vi "FuncVI_Sub - Format to string.vi"(5 "InstanceRef":T2, 7 "format error enabled":bool, 9 "arg list":T1[](array[typedef]) {"num" format="%.2f"}) -> (0 "error out":bool, 3 "result":T1 {"num" format="%.2f"})   [LabVIEW 2021]
doc: "::: CalcExpress Toolkit :::\nCopyright (c) 2000-2026 Konstantin Shifershteyn. All rights reserved."
uses:
  cetypes.llb/CalcExpress Function Argument Info.ctl
  cetypes.llb/CalcExpress Instance RefNum.ctl
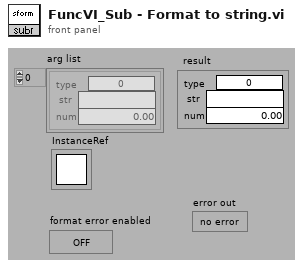
[diagram p1: front panel]
types:
  T1 = typedef "CalcExpress Function Argument Info.ctl" = cluster{"type":u32, "str":string, "num":dbl}
  T2 = typedef "CalcExpress Instance RefNum.ctl" = refnum<k1>
  T3 = enum32{"String", "DBL Number", "identifier", "1D Array of DBL", "2D Array of DBL", "CDB Number", "1D Array of CDB", "2D Array of CDB", "1D Array of String", "2D Array of String", "Unknown data type"}
  T4 = cluster{"type":enum32{"String", "DBL Number", "identifier", "1D Array of DBL", "2D Array of DBL", "CDB Number", "1D Array of CDB", "2D Array of CDB", "1D Array of String", "2D Array of String", "Unknown data type"}, string, "return value":dbl}
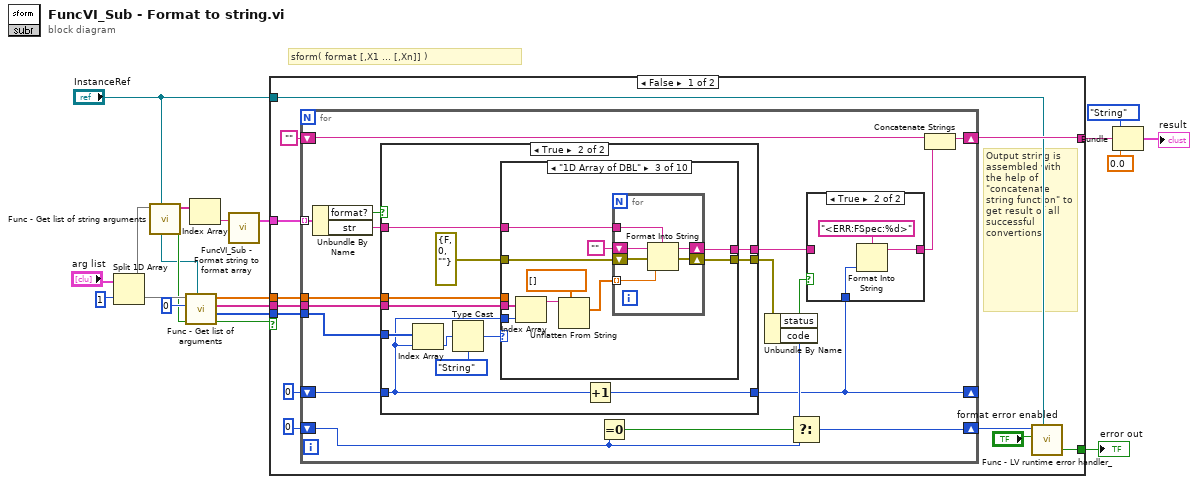
[diagram p0: block diagram]
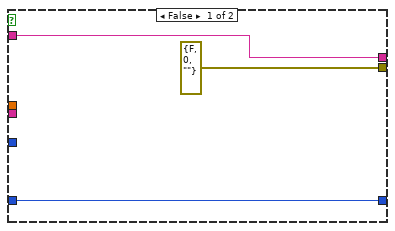
[diagram p3: hidden frame]
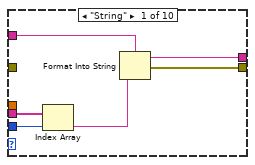
[diagram p4: hidden frame]
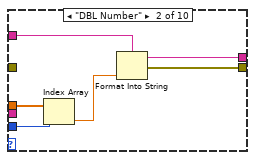
[diagram p5: hidden frame]
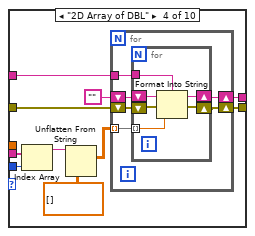
[diagram p6: hidden frame]
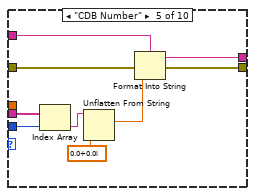
[diagram p7: hidden frame]
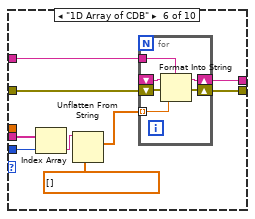
[diagram p8: hidden frame]
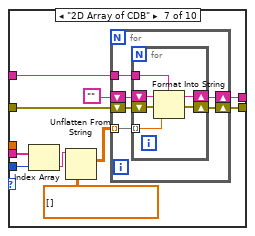
[diagram p9: hidden frame]
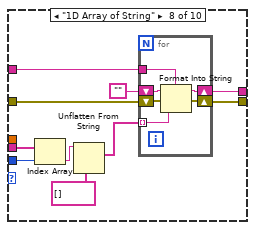
[diagram p10: hidden frame]
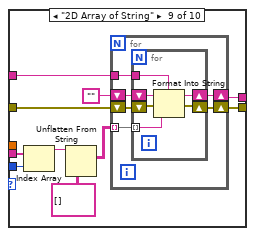
[diagram p11: hidden frame]
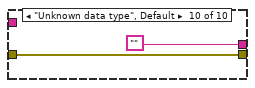
[diagram p12: hidden frame]
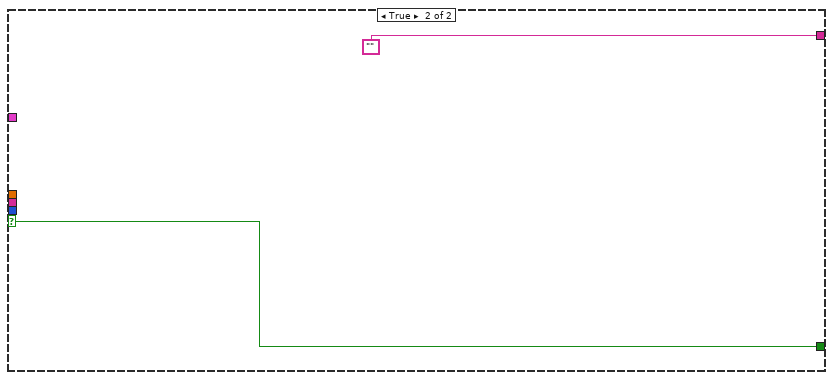
[diagram p13: hidden frame]
diagram:
  # "sform( format [,X1 ... [,Xn]] )"
  n1 = Split 1D Array(array="arg list", index=1) -> (first subarray=w17:T1[], second subarray=w16:T1[])
  n2 = call "Func - Get list of string arguments.vi"("InstanceRef"="InstanceRef", "arg list"=w17) -> ("error out"=w7:bool, "val list"=w5:string[])  [unwired: 6 in]
  n3 = call "Func - Get list of arguments.vi"("InstanceRef"="InstanceRef", "error in"=w7, "min arg num"=0 ("min args num"), "arg list"=w16) -> ("error out"=w6:bool, "type list"=w13:u32[], "str list"=w14:string[], "num list"=w2:dbl[])  [unwired: 4 in]
  n4 = Index Array(array=w5) -> (element=w4:string)  [unwired: 1 in]
  n5 = call "FuncVI_Sub - Format string to format array.vi"("format string"=w4) -> ("formats"=w3:cluster{"str":string, "format?":bool}[])  [unwired: 1 in, 1 out]
  n6 = case shown="False" w6 {
    selector: w6 -> [_ w205]
    tunnel: w2 -> [w31 _]
    tunnel: w14 -> [w30 _]
    tunnel: w13 -> [w28 _]
    tunnel: [w23 w205] -> w12
    tunnel: [w29 "" ("Empty String Constant")] -> w10
    tunnel: w3 -> [w25 _]
    tunnel: "InstanceRef" -> [w21 _]
    frame False {
      # "Output string is assembled with the help of \"concatenate string function\" to get result of all successful convertions."
      n7 = for {
        shift-right: [w39] -> w29
        shift-left: "" ("Empty String Constant") -> [w38]
        tunnel: w31 -> [w49]
        tunnel: w30 -> [w48]
        tunnel: w28 -> [w47]
        tunnel: w25 -> [w46] mode=indexing
        shift-right: [w34] -> _
        shift-left: 0 -> [w43]
        shift-right: [w40] -> w20
        shift-left: 0 -> [w41]
        n8 = Unbundle By Name(w46) -> ("format?"=w44:bool, "str"=w45:string)
        n9 = case shown="True" w44 {
          tunnel: w49 -> [_ w68]
          tunnel: w48 -> [_ w67]
          tunnel: w47 -> [_ w63]
          tunnel: [errorcluster {"status"=FALSE, "code"=0, "source"=""} ("error IO") w66] -> w42
          tunnel: w45 -> [w54 w65]
          tunnel: w43 -> [w56 w61]
          tunnel: [w56 w64] -> w34
          tunnel: [w54 w59] -> w33
          frame False {
          }
          frame True {
            n10 = Index Array(array=w63, index=w61) -> (element=w62:u32)
            n11 = Type Cast(type=T3."String", x=w62) -> (*(type *) &x=w58:T3)
            n12 = case shown="\"1D Array of DBL\"" w58 {
              tunnel: w68 -> [_ w77 _ _ _ _ _ _ _ _]
              tunnel: w67 -> [w74 _ w84 w99 w123 w136 w152 w174 w185 _]
              tunnel: [w73 w80 w86 w101 w127 w131 w147 w169 w186 "" ("Empty String Constant")] -> w59
              tunnel: [w72 w79 w88 w102 w126 w133 w148 w171 w187 w204] -> w66
              tunnel: w65 -> [w71 w78 w82 w104 w125 w128 w144 w168 w182 _]
              tunnel: errorcluster {"status"=FALSE, "code"=0, "source"=""} ("error IO") -> [_ _ w89 w103 w124 w134 w149 w172 w188 w204]
              tunnel: w61 -> [w69 w76 w85 w98 w119 w129 w145 w166 w184 _]
              frame "String" {
                n13 = Index Array(array=w74, index=w69) -> (element=w70:string)
                n14 = Format Into String(format string=w71, w70) -> (resulting string=w73:string, error out=w72:errorcluster)  [unwired: 2 in]
              }
              frame "DBL Number" {
                n15 = Index Array(array=w77, index=w76) -> (element=w75:dbl)
                n16 = Format Into String(format string=w78, w75) -> (resulting string=w80:string, error out=w79:errorcluster)  [unwired: 2 in]
              }
              frame "1D Array of DBL" {
                n17 = Index Array(array=w84, index=w85) -> (element=w83:string)
                n18 = Unflatten From String(type=dbl[] [] ("num list"), binary string=w83) -> (value=w87:dbl[])  [unwired: 3 in, 2 out]
                n19 = for {
                  tunnel: w87 -> [w96] mode=indexing
                  shift-right: [w93] -> w86
                  shift-left: "" ("Empty String Constant") -> [w92]
                  shift-right: [w94] -> w88
                  shift-left: w89 -> [w95]
                  tunnel: w82 -> [w91]
                  n20 = Format Into String(format string=w91, initial string=w92, error in=w95, w96) -> (resulting string=w93:string, error out=w94:errorcluster)
                }
              }
              frame "2D Array of DBL" {
                n21 = Index Array(array=w99, index=w98) -> (element=w100:string)
                n22 = Unflatten From String(type=dbl[][] [] ("num list"), binary string=w100) -> (value=w105:dbl[][])  [unwired: 3 in, 2 out]
                n23 = for {
                  tunnel: w105 -> [w112] mode=indexing
                  tunnel: w104 -> [w111]
                  shift-right: [w109] -> w102
                  shift-left: w103 -> [w110]
                  shift-right: [w108] -> w101
                  shift-left: "" ("Empty String Constant") -> [w107]
                  n24 = for {
                    tunnel: w112 -> [w118] mode=indexing
                    shift-right: [w114] -> w108
                    shift-left: w107 -> [w113]
                    shift-right: [w116] -> w109
                    shift-left: w110 -> [w117]
                    tunnel: w111 -> [w115]
                    n25 = Format Into String(format string=w115, initial string=w113, error in=w117, w118) -> (resulting string=w114:string, error out=w116:errorcluster)
                  }
                }
              }
              frame "CDB Number" {
                n26 = Index Array(array=w123, index=w119) -> (element=w120:string)
                n27 = Unflatten From String(type=cdb 0.0+0.0i, binary string=w120) -> (value=w122:cdb)  [unwired: 3 in, 2 out]
                n28 = Format Into String(format string=w125, error in=w124, w122) -> (resulting string=w127:string, error out=w126:errorcluster)  [unwired: 1 in]
              }
              frame "1D Array of CDB" {
                n29 = Index Array(array=w136, index=w129) -> (element=w130:string)
                n30 = Unflatten From String(type=cdb[] [] ("num list"), binary string=w130) -> (value=w132:cdb[])  [unwired: 3 in, 2 out]
                n31 = for {
                  tunnel: w132 -> [w142] mode=indexing
                  shift-right: [w138] -> w131
                  shift-left: _ -> [w139]
                  shift-right: [w140] -> w133
                  shift-left: w134 -> [w141]
                  tunnel: w128 -> [w137]
                  n32 = Format Into String(format string=w137, initial string=w139, error in=w141, w142) -> (resulting string=w138:string, error out=w140:errorcluster)
                }
              }
              frame "2D Array of CDB" {
                n33 = Index Array(array=w152, index=w145) -> (element=w146:string)
                n34 = Unflatten From String(type=cdb[][] [] ("num list"), binary string=w146) -> (value=w150:cdb[][])  [unwired: 3 in, 2 out]
                n35 = for {
                  tunnel: w150 -> [w158] mode=indexing
                  shift-right: [w156] -> w148
                  shift-left: w149 -> [w157]
                  shift-right: [w155] -> w147
                  shift-left: "" ("Empty String Constant") -> [w154]
                  tunnel: w144 -> [w153]
                  n36 = for {
                    tunnel: w158 -> [w164] mode=indexing
                    shift-right: [w161] -> w155
                    shift-left: w154 -> [w160]
                    shift-right: [w162] -> w156
                    shift-left: w157 -> [w163]
                    tunnel: w153 -> [w159]
                    n37 = Format Into String(format string=w159, initial string=w160, error in=w163, w164) -> (resulting string=w161:string, error out=w162:errorcluster)
                  }
                }
              }
              frame "1D Array of String" {
                n38 = Index Array(array=w174, index=w166) -> (element=w167:string)
                n39 = Unflatten From String(type=string[] [] ("num list"), binary string=w167) -> (value=w170:string[])  [unwired: 3 in, 2 out]
                n40 = for {
                  tunnel: w170 -> [w180] mode=indexing
                  shift-right: [w176] -> w169
                  shift-left: "" ("Empty String Constant") -> [w177]
                  shift-right: [w178] -> w171
                  shift-left: w172 -> [w179]
                  tunnel: w168 -> [w175]
                  n41 = Format Into String(format string=w175, initial string=w177, error in=w179, w180) -> (resulting string=w176:string, error out=w178:errorcluster)
                }
              }
              frame "2D Array of String" {
                n42 = Index Array(array=w185, index=w184) -> (element=w183:string)
                n43 = Unflatten From String(type=string[][] [] ("num list"), binary string=w183) -> (value=w189:string[][])  [unwired: 3 in, 2 out]
                n44 = for {
                  tunnel: w189 -> [w196] mode=indexing
                  shift-right: [w194] -> w187
                  shift-left: w188 -> [w195]
                  shift-right: [w193] -> w186
                  shift-left: "" ("Empty String Constant") -> [w192]
                  tunnel: w182 -> [w191]
                  n45 = for {
                    tunnel: w196 -> [w202] mode=indexing
                    shift-right: [w199] -> w193
                    shift-left: w192 -> [w198]
                    shift-right: [w200] -> w194
                    shift-left: w195 -> [w201]
                    tunnel: w191 -> [w197]
                    n46 = Format Into String(format string=w197, initial string=w198, error in=w201, w202) -> (resulting string=w199:string, error out=w200:errorcluster)
                  }
                }
              }
              frame "Unknown data type", Default {
              }
            }
            n47 = Increment(x=w61) -> (x+1=w64:i32)
          }
        }
        n48 = Equal To 0?(x=w41) -> (x = 0?=w37:bool)
        n49 = Unbundle By Name(w42) -> ("status"=w35:bool, "code"=w36:i32)
        n50 = Select(t=w36, s=w37, f=w41) -> (s? t:f=w40:i32)
        n51 = case shown="True" w35 {
          tunnel: w33 -> [w50 _]
          tunnel: [w50 w52] -> w32
          tunnel: w34 -> [_ w51]
          frame False {
          }
          frame True {
            n52 = Format Into String(format string="<ERR:FSpec:%d>", w51) -> (resulting string=w52:string)  [unwired: 2 in, 1 out]
          }
        }
        n53 = Concatenate Strings(w38, w32) -> (w39:string)
      }
      n54 = call "Func - LV runtime error handler_.vi"("InstanceRef"=w21, "Gen CE error?"="format error enabled", "LabVIEW error code"=w20) -> ("error out"=w23:bool)  [unwired: 8 in]
    }
    frame True {
    }
  }
  "error out" <- w12
  n55 = Bundle("type"=T3."String", w10, "return value"=0.0) -> (→"result":T4)  [unwired: 1 in]
